vi "RemoteVI Open Server Loop.vi"(1 "loop VI":path, 11 "error in":errorcluster) -> (4 "Server Loop":refnum<vi>, 15 "error out":errorcluster)   [LabVIEW 2020, in "RemoteVI.lvlib"]
doc: "Opens a new instance of RemoteVI Server Loop.vi, found next to this VI (both live in source\\Server): the Server Loop is reentrant (preallocated clone), and Open VI Reference with option 0x08 (prepare for reentrant run) returns a reference to a clone of its own, so every share of this LabVIEW application instance runs its own loop. loop VI (not empty) opens that VI instead the same way - RemoteVI Start Landing Page.vi opens the reentrant RemoteVI Landing Server.vi. Nothing is opened on an incoming error."
uses:
  RemoteVI.lvlib
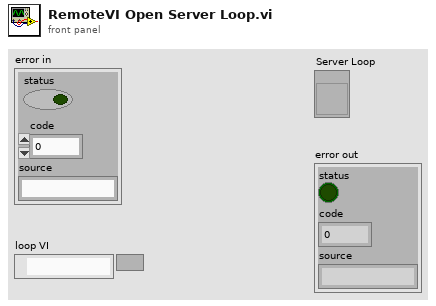
[diagram p1: front panel]
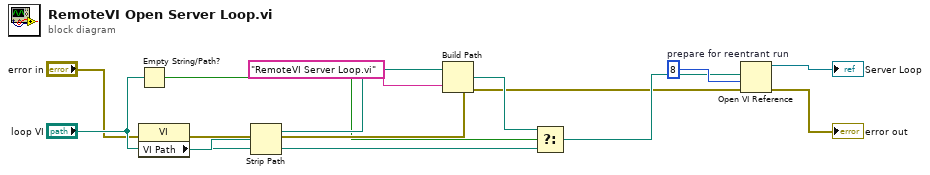
[diagram p0: block diagram]
diagram:
  w10 = u32 8  # prepare for reentrant run
  n1 = Empty String/Path?(string/path="loop VI") -> (empty?=w3:bool)
  n2 = property class="VI"(error in="error in") -> (error out=w4:errorcluster, "VI Path"=w5:path)  [unwired: 1 in, 1 out]
  n3 = Strip Path(path=w5) -> (stripped path=w6:path)  [unwired: 1 out]
  n4 = Build Path(base path=w6, name or relative path="RemoteVI Server Loop.vi") -> (appended path=w8:path)
  n5 = Select(t=w8, s=w3, f="loop VI") -> (s? t:f=w9:path)
  n6 = Open VI Reference(vi path=w9, options=w10, error in (no error)=w4) -> (vi reference=→"Server Loop":refnum<vi>, error out=→"error out":errorcluster)  [unwired: 3 in]
